vi "Create Sysdef Tree Labels.vi"(6 "first call":bool, 7 "Autocreate Rx timestamp chans?":bool, 8 "error in":errorcluster, 9 "Labels":T2[](array[typedef]), 10 "Section Ptr":T1 format="%.0x", 11 "direction":T6(ring)) -> (0 "error out":errorcluster)   [LabVIEW 2015, in "AIT 429 System Explorer.lvlib"]
uses:
  AIT 429 System Explorer.lvlib
  Controls/AIT_Label.ctl
  Controls/AIT_Word.ctl
  Controls/ARINCParam.ctl
  Shared/Controls and Global/TransferType.ctl
  <vilib>/NI Veristand/Custom Device API/Custom Device Item Ref.ctl
  <vilib>/NI Veristand/Custom Device API/Custom Device Channel.ctl
  <vilib>/NI Veristand/Custom Device API/Custom Device Channel Type.ctl
  Shared/Controls and Global/Global.vi
  <vilib>/NI Veristand/Custom Device API/Custom Device API.lvlib
  Shared/AIT 429 Shared.lvlib
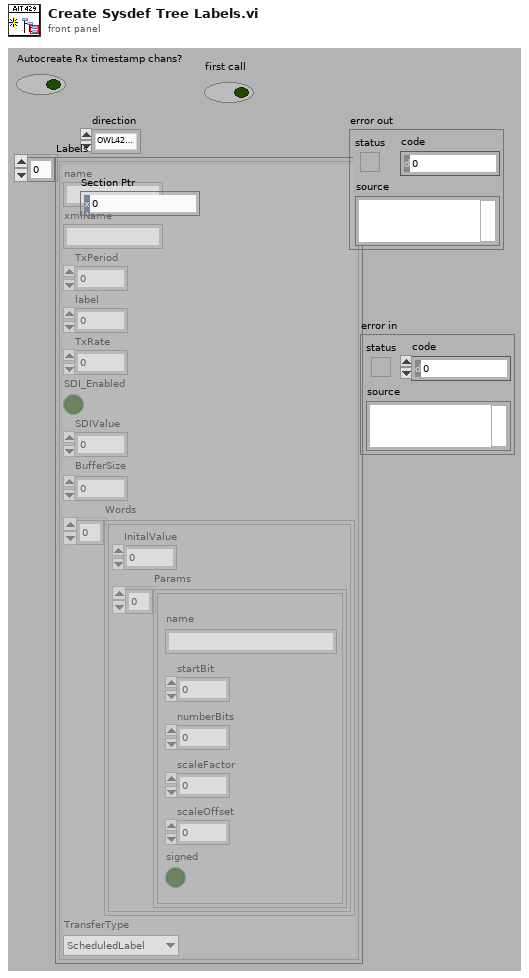
[diagram p1: front panel]
types:
  T1 = typedef "Custom Device API.lvlib/Custom Device Item Ref.ctl" = u64
  T2 = typedef "AIT 429 System Explorer.lvlib/AIT_Label.ctl" = cluster{"name":string, "xmlName":string, "TxPeriod":u32, "label":u32, "TxRate":dbl, "SDI_Enabled":bool, "SDIValue":u8, "BufferSize":u32, "Words":T3[], "TransferType":T5}
  T3 = typedef "AIT 429 System Explorer.lvlib/AIT_Word.ctl" = cluster{"InitalValue":u32, "Params":T4[]}
  T4 = typedef "AIT 429 System Explorer.lvlib/ARINCParam.ctl" = cluster{"name":string, "startBit":i32, "numberBits":i32, "scaleFactor":dbl, "scaleOffset":dbl, "signed":bool}
  T5 = typedef "AIT 429 Shared.lvlib/TransferType.ctl" = enum16{"ScheduledLabel", "Acyclic", "Block", "Strobe"}
  T6 = enum16{"OWL429_DIRECTION_RX", "OWL429_DIRECTION_TX"}
  T7 = typedef "Custom Device API.lvlib/Custom Device Channel.ctl" = cluster{"Type":T8, "Units":string, "Default Value":dbl, "Faultable":bool, "Scalable":bool}
  T8 = typedef "Custom Device API.lvlib/Custom Device Channel Type.ctl" = enum16{"Input", "Output"}
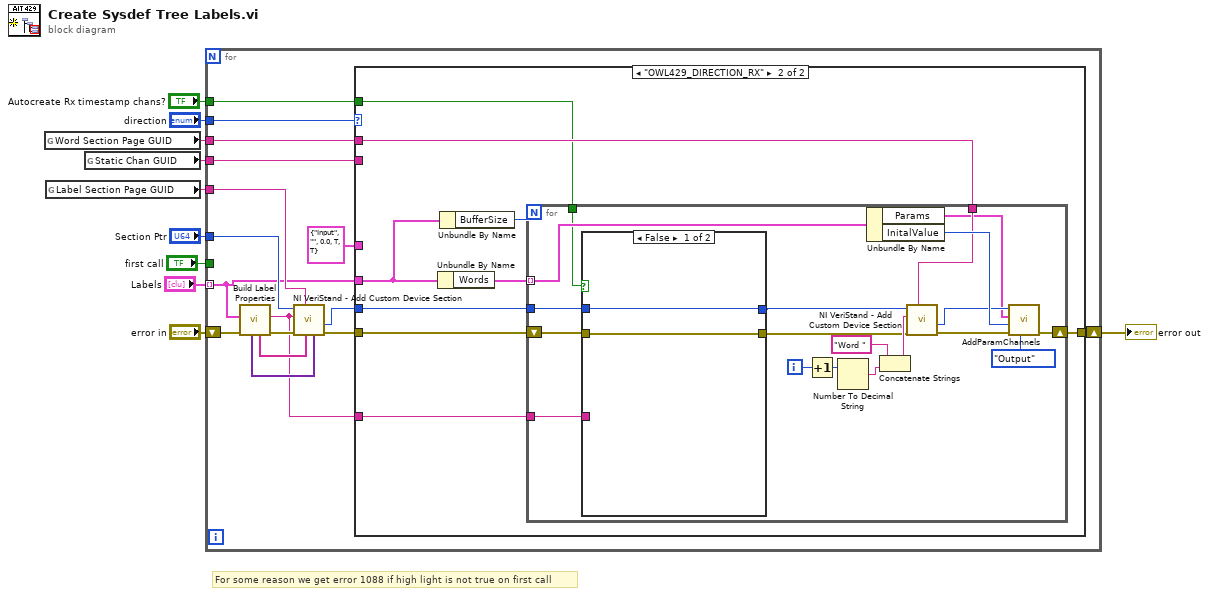
[diagram p0: block diagram]
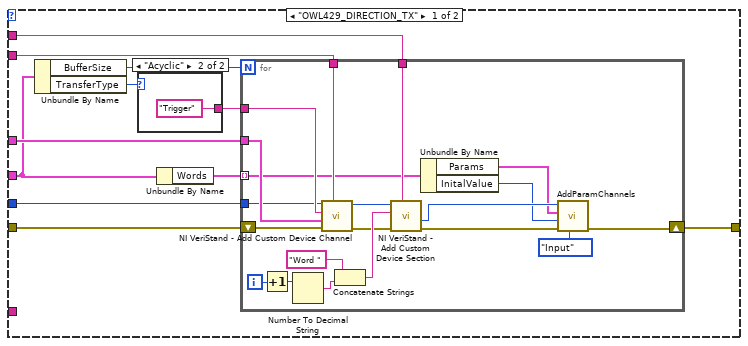
[diagram p2: hidden frame]
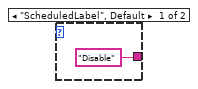
[diagram p3: hidden frame]
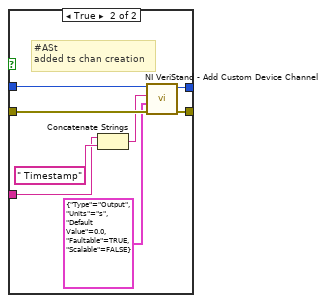
[diagram p4: hidden frame]
diagram:
  # "For some reason we get error 1088 if high light is not true on first call"
  n1 = global read "Global.vi" "Word Section Page GUID"() -> (w5:string)
  n2 = global read "Global.vi" "Label Section Page GUID"() -> (w7:string)
  n3 = global read "Global.vi" "Static Chan GUID"() -> (w6:string)
  n4 = for {
    shift-right: [w23] -> w4
    shift-left: "error in" -> [w15]
    tunnel: "Section Ptr" -> [w25]
    tunnel: "Labels" -> [w17] mode=indexing
    tunnel: "direction" -> [w22]
    tunnel: w7 -> [w20]
    tunnel: w6 -> [w19]
    tunnel: w5 -> [w16]
    tunnel: "first call" -> [_]
    tunnel: "Autocreate Rx timestamp chans?" -> [w12]
    n5 = call "Build Label Properties.vi"("error in (no error)"=w15, "Labels"=w17) -> ("error out"=w14:errorcluster, "name"=w11:string, "Prop Names"=w24:string[], "Prop Values"=w26:variant[])  [unwired: 6 in]
    n6 = call <vilib>:"NI VeriStand - Add Custom Device Section.vi"("Property Values"=w26, "Property names"=w24, "GUID (Default Section)"=w20, "error in (no error)"=w14, "Section Name"=w11, "Parent Ref in"=w25) -> ("error out"=w13:errorcluster, "Section Ptr"=w18:T1)  [unwired: 2 in, 2 out]
    n7 = case shown="\"OWL429_DIRECTION_RX\"" w22 {
      tunnel: w13 -> [w34 w68]
      tunnel: w18 -> [w33 w65]
      tunnel: [w37 w67] -> w23
      tunnel: T7 {"Type"=enum."Input", "Units"="", "Default Value"=0.0, "Faultable"=TRUE, "Scalable"=TRUE} ("Channel") -> [w36 _]
      tunnel: w19 -> [w35 _]
      tunnel: w17 -> [w30 w66]
      tunnel: w16 -> [w32 w64]
      tunnel: w12 -> [_ w61]
      tunnel: w11 -> [_ w60]
      frame "OWL429_DIRECTION_TX" {
        n8 = Unbundle By Name(w30) -> ("BufferSize"=w29:u32, "TransferType"=w28:T5)
        n9 = case shown="\"Acyclic\"" w28 {
          tunnel: ["Disable" ("Channel Name") "Trigger" ("Static Chan GUID")] -> w27
          frame "ScheduledLabel", Default {
          }
          frame "Acyclic" {
          }
        }
        n10 = Unbundle By Name(w30) -> ("Words"=w31:T3[])
        n11 = for {
          N: w29 -> [_]
          tunnel: w36 -> [w59]
          tunnel: w27 -> [w58]
          tunnel: w35 -> [w57]
          tunnel: w33 -> [w50]
          tunnel: w31 -> [w47] mode=indexing
          shift-right: [w43] -> w37
          shift-left: w34 -> [w49]
          tunnel: w32 -> [w52]
          i -> [w54]
          n12 = Increment(x=w54) -> (x+1=w55:i32)
          n13 = Number To Decimal String(number=w55) -> (decimal integer string=w56:string)  [unwired: 1 in]
          n14 = call <vilib>:"NI VeriStand - Add Custom Device Channel.vi"("GUID (Default Channel)"=w57, "error in (no error)"=w49, "Channel"=w59, "Channel Name"=w58, "Parent Ref in"=w50) -> ("error out"=w41:errorcluster, "Parent Ref out"=w48:T1)  [unwired: 3 in, 2 out]
          n15 = Concatenate Strings("Word " ("string"), w56) -> (w51:string)
          n16 = call <vilib>:"NI VeriStand - Add Custom Device Section.vi"("GUID (Default Section)"=w52, "error in (no error)"=w41, "Section Name"=w51, "Parent Ref in"=w48) -> ("error out"=w42:errorcluster, "Section Ptr"=w46:T1)  [unwired: 4 in, 2 out]
          n17 = Unbundle By Name(w47) -> ("Params"=w40:T4[], "InitalValue"=w45:u32)
          n18 = call "AddParamChannels.vi"("Type"=Custom_Device_Channel_Type."Input", "error in"=w42, "Initial Value"=w45, "Parameters to add"=w40, "Node Ref In"=w46) -> ("error out"=w43:errorcluster)  [unwired: 5 in, 1 out]
        }
      }
      frame "OWL429_DIRECTION_RX" {
        n19 = Unbundle By Name(w66) -> ("Words"=w63:T3[])
        n20 = Unbundle By Name(w66) -> ("BufferSize"=w62:u32)
        n21 = for {
          N: w62 -> [_]
          tunnel: w65 -> [w70]
          tunnel: w63 -> [w86] mode=indexing
          shift-right: [w71] -> w67
          shift-left: w68 -> [w73]
          tunnel: w64 -> [w84]
          tunnel: w61 -> [w76]
          tunnel: w60 -> [w74]
          i -> [w83]
          n22 = case shown="False" w76 {
            tunnel: w73 -> [w89 w97]
            tunnel: [w89 w94] -> w72
            tunnel: w74 -> [_ w92]
            tunnel: w70 -> [w88 w91]
            tunnel: [w88 w90] -> w69
            frame False {
            }
            frame True {
              # "#ASt\nadded ts chan creation"
              n23 = Concatenate Strings(w92, " Timestamp" ("string")) -> (w96:string)
              n24 = call <vilib>:"NI VeriStand - Add Custom Device Channel.vi"("error in (no error)"=w97, "Channel"=T7 {"Type"=enum."Output", "Units"="s", "Default Value"=0.0, "Faultable"=TRUE, "Scalable"=FALSE}, "Channel Name"=w96, "Parent Ref in"=w91) -> ("error out"=w94:errorcluster, "Parent Ref out"=w90:T1)  [unwired: 4 in, 2 out]
            }
          }
          n25 = Increment(x=w83) -> (x+1=w82:i32)
          n26 = Number To Decimal String(number=w82) -> (decimal integer string=w81:string)  [unwired: 1 in]
          n27 = Unbundle By Name(w86) -> ("Params"=w77:T4[], "InitalValue"=w87:u32)
          n28 = Concatenate Strings("Word " ("string"), w81) -> (w75:string)
          n29 = call <vilib>:"NI VeriStand - Add Custom Device Section.vi"("GUID (Default Section)"=w84, "error in (no error)"=w72, "Section Name"=w75, "Parent Ref in"=w69) -> ("error out"=w85:errorcluster, "Section Ptr"=w78:T1)  [unwired: 4 in, 2 out]
          n30 = call "AddParamChannels.vi"("Type"=Custom_Device_Channel_Type."Output", "error in"=w85, "Initial Value"=w87, "Parameters to add"=w77, "Node Ref In"=w78) -> ("error out"=w71:errorcluster)  [unwired: 5 in, 1 out]
        }
      }
    }
  }
  "error out" <- w4
